vi "Disable VIO.vi"(0 "instrument handle":refnum<k15>, 5 "Bus Number":i32, 11 "error in":errorcluster) -> (4 "instrument handle out":refnum<k15>, 15 "error out":errorcluster)   [LabVIEW 2018, in "MIPI RFFE API.lvlib"]
uses:
  MIPI RFFE API.lvlib
  <instrlib>/niDigital/niDigital.llb/niDigital Selected Function.ctl
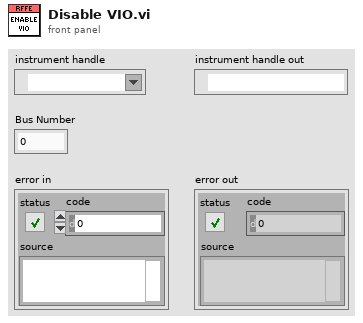
[diagram p1: front panel]
types:
  T1 = typedef "niDigital Selected Function.ctl" = i32
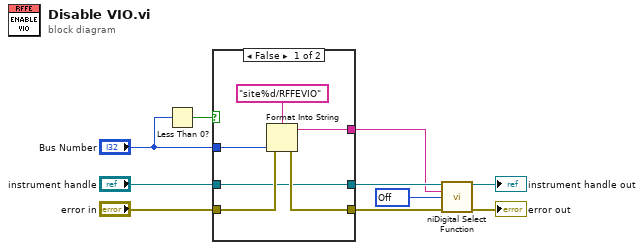
[diagram p0: block diagram]
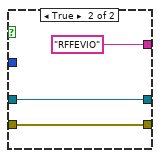
[diagram p2: hidden frame]
diagram:
  w1 = T1 1102 items=["Digital"=1100, "PPMU"=1101, "Off"=1102, "Disconnect"=1103] ("function")
  n1 = Less Than 0?(x="Bus Number") -> (x < 0?=w5:bool)
  n2 = case shown="False" w5 {
    tunnel: "error in" -> [w13 w18]
    tunnel: [w14 "RFFEVIO" ("channel list")] -> w2
    tunnel: "Bus Number" -> [w15 _]
    tunnel: [w12 w18] -> w4
    tunnel: "instrument handle" -> [w11 w17]
    tunnel: [w11 w17] -> w3
    frame False {
      n3 = Format Into String(format string="site%d/RFFEVIO" ("channel list"), error in=w13, w15) -> (resulting string=w14:string, error out=w12:errorcluster)  [unwired: 1 in]
    }
    frame True {
    }
  }
  n4 = call <instrlib>:"niDigital Select Function.vi"("instrument handle"=w3, "channel list"=w2, "function"=w1, "error in"=w4) -> ("instrument handle out"=→"instrument handle out":refnum<k15>, "error out"=→"error out":errorcluster)  [unwired: 10 in]
